vi "update.description.request.vi"(8 "error in":errorcluster, 11 "Description":string) -> (0 "error out":errorcluster, 1 "Request":string)   [LabVIEW 2020, in "Run.lvclass"]
uses:
  Run.lvclass
  <vilib>/JDP Science/JSONtext/support/Format JSON Object.vi
  Run.lvclass/Run.ctl
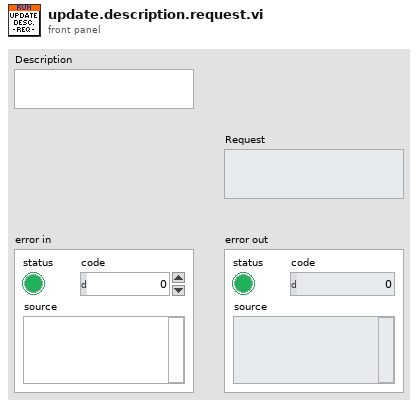
[diagram p1: front panel]
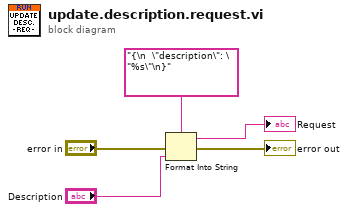
[diagram p0: block diagram]
diagram:
  n1 = Format Into String(format string="{\n  \"description\": \"%s\"\n}", error in="error in", "Description") -> (resulting string=→"Request":string, error out=→"error out":errorcluster)  [unwired: 1 in]
